vi "configuration UI.vi"() -> ()   [LabVIEW 2013, in "EIP Tags editor node.lvclass"]
uses:
  EIP Tags editor node.lvclass
  <vilib>/NI/Configuration Framework/Node/NodeRef.ctl
  <vilib>/NI/Configuration Framework/Node/NISE_CEF_Node.lvclass
  <vilib>/NI/AMC/Message Queue.ctl
  <vilib>/NI/AMC/Message.ctl
  <vilib>/NI/Tools/Keyed Array/KeyedArray.ctl
  <vilib>/NI/Configuration Framework/Node/UserEventRef.ctl
  <vilib>/NI/Configuration Framework/Controls/EventCluster.ctl
  <vilib>/NI/DCAF UI Toolkit/Controls/Configure.ctl
  <vilib>/NI/DCAF UI Toolkit/Controls/Add.ctl
  <vilib>/NI/DCAF UI Toolkit/Controls/Remove.ctl
  <vilib>/NI/DCAF UI Toolkit/Controls/Import.ctl
  <vilib>/Utility/miscctls.llb/LVPositionTypeDef.ctl
  <vilib>/NI/DCAF/Tag Editor Core/Configuration Editor/Classes/Engine Parent/Engine Parent Editor Node.lvclass
  <vilib>/NI/Tag Bus/tag/tag descriptor.lvclass
  <vilib>/NI/Tag Bus/tag/Data Type.ctl
  <vilib>/NI/Module Execution Interface/Engine Configuration/engine configuration.lvclass
  configuration/EIP Tags Configuration.lvclass
  <vilib>/NI/Tag Bus/tag/tag descriptor.lvclass/tag descriptor.ctl
  EIP Tags editor node.lvclass/EIP Tags editor node.ctl
  configuration/eip tag definition.ctl
  configuration/eip tag types.ctl
  <vilib>/NI/Configuration Framework/serializable configuration/NISE_CEF_serializable configuration.lvclass/NISE_CEF_serializable configuration.ctl
  <vilib>/NI/Tag Bus/tag/write tag name.vi
  <vilib>/NI/Tag Bus/tag/write data type.vi
  <vilib>/NI/DCAF/Tag Editor Core/Configuration Editor/Classes/Module editor node/Read Module Configuration.vi
  <vilib>/Utility/LVClass/Get LV Class Name.vi
  <vilib>/NI/Configuration Framework/error generator/NISE_error generator.vi
  <vilib>/NI/Tag Bus Module Framework/module configuration/TBM module configuration.lvclass
  <vilib>/NI/Configuration Framework/NISE_CEF_TreeControl.lvlib
  <vilib>/NI/DCAF/Tag Editor Core/Configuration Editor/Classes/Module editor node/module editor node.lvclass
  <vilib>/NI/Configuration Framework/serializable configuration/NISE_CEF_serializable configuration.lvclass
  <vilib>/NI/DCAF UI Toolkit/Controls/DCAF UI Elements.lvlib
  <vilib>/NI/Tools/Keyed Array/Tools_KeyedArray.lvlib
  <vilib>/NI/AMC/AMC.lvlib
panel:
  in  "Top Level Tab Control":enum32{"EIP Tags", "Channels"}(tab)
  in  "EIP tags":i32(listbox)
  in  "Add EIPT":T1
  in  "Remove EIPT":T2
  in  "configure EIPT":T3
  in  "generate from csv":T4
  in  "settings":T3
  in  "channel":i32(listbox)
  in  "Add Button":T1
  in  "Remove Button":T2
  in  "hidden_add":bool
  in  "user event":T5
  in  "main queue":T6
  in  "node ref":T7
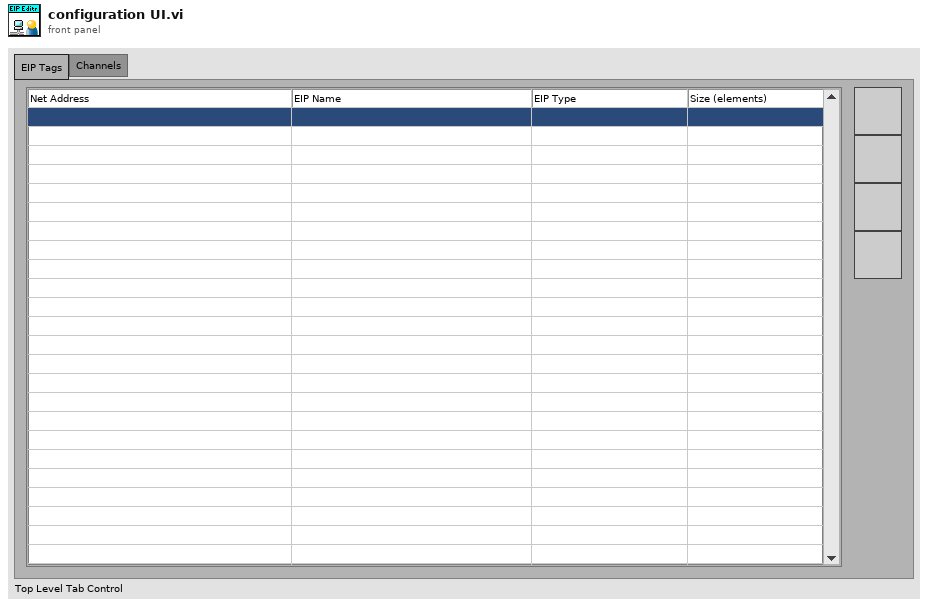
[diagram p1: front panel]
types:
  T1 = typedef "DCAF UI Elements.lvlib/Add.ctl" = bool
  T2 = typedef "DCAF UI Elements.lvlib/Remove.ctl" = bool
  T3 = typedef "DCAF UI Elements.lvlib/Configure.ctl" = bool
  T4 = typedef "DCAF UI Elements.lvlib/Import.ctl" = bool
  T5 = typedef "NISE_CEF_Node.lvclass/UserEventRef.ctl" = refnum<user-event>
  T6 = typedef "AMC.lvlib/Message Queue.ctl" = refnum<queue>
  T7 = typedef "NISE_CEF_Node.lvclass/NodeRef.ctl" = refnum<data-value>
  T8 = typedef "LVPositionTypeDef.ctl" = cluster{"Left":i32, "Top":i32}
  T9 = typedef "NISE_CEF_TreeControl.lvlib/EventCluster.ctl" = cluster{"command":string, "data":string}
  T10 = typedef "tag bus.lvlib/tag descriptor.lvclass/Data Type.ctl" = enum16{"Double", "Single", "I64", "I32", "I16", "I8", "U64", "U32", "U16", "U8", "Boolean", "String", "Array of Double", "Array of Single", "Array of I64", "Array of I32", "Array of I16", "Array of I8", "Array of U64", "Array of U32", "Array of U16", "Array of U8", "Array of Boolean", "Array of String"}
  T11 = typedef "EIP Tags Configuration.lvclass/eip tag definition.ctl" = cluster{"eip tag types":T12, "unique tag name":string, "Number of Elements":u32}
  T12 = typedef "EIP Tags Configuration.lvclass/eip tag types.ctl" = enum16{"SINT", "INT", "DINT", "REAL", "BOOL", "STRING"}
  T13 = typedef "EIP Tags editor node.lvclass/table line.ctl" = cluster{"eip channel":refnum<class "EIP Tags Channel.lvclass">, "tag name":string}
  T14 = typedef "LVPoint32TypeDef.ctl" = cluster{"Horizontal":i32, "Vertical":i32}
  T15 = typedef "LVRowAndColumnTypeDef.ctl" = cluster{"Row":i32, "Column":i32}
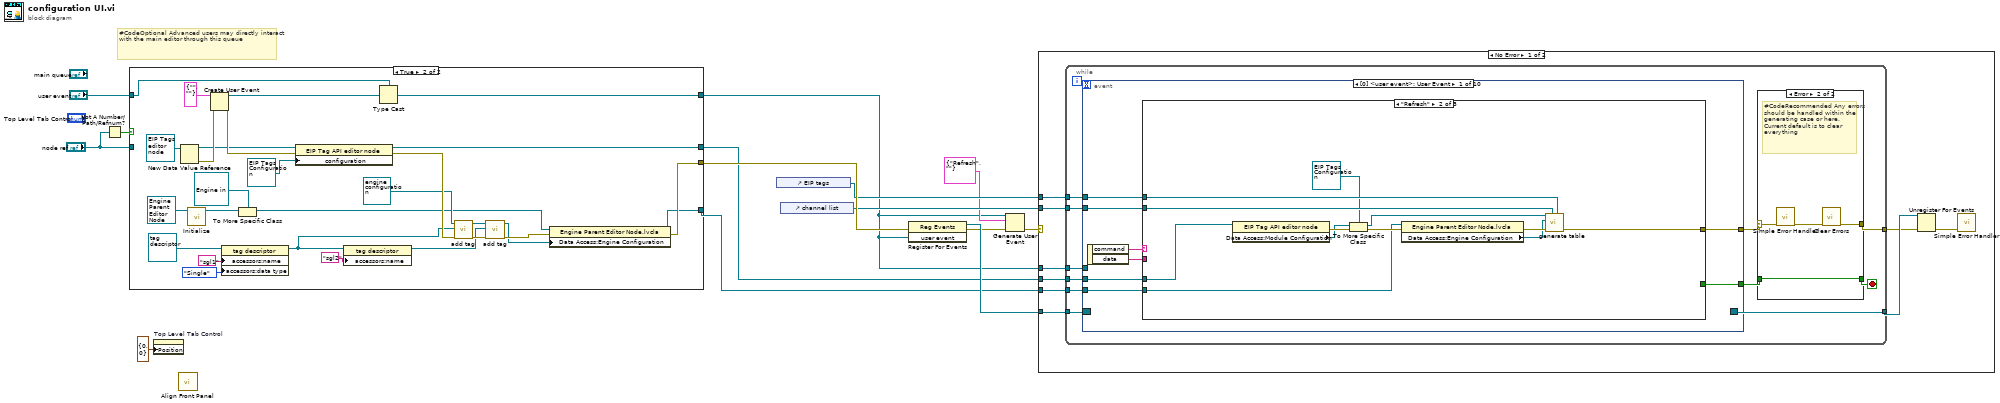
[diagram p0: block diagram]
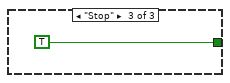
[diagram p4: hidden frame]
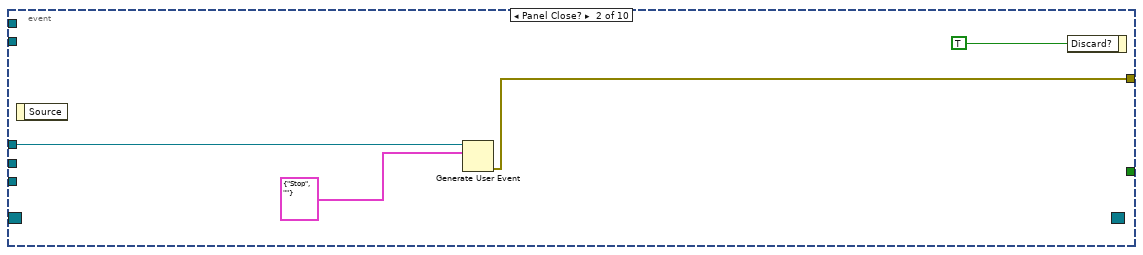
[diagram p5: hidden frame]
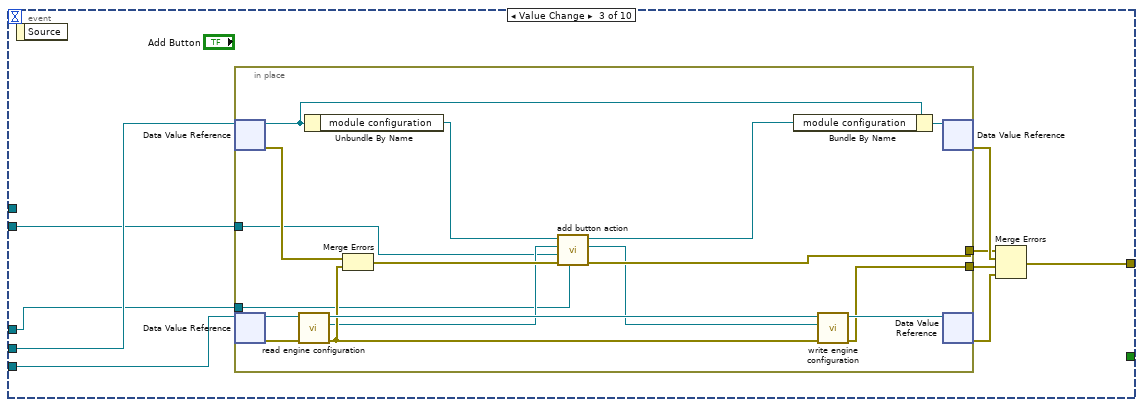
[diagram p6: hidden frame]
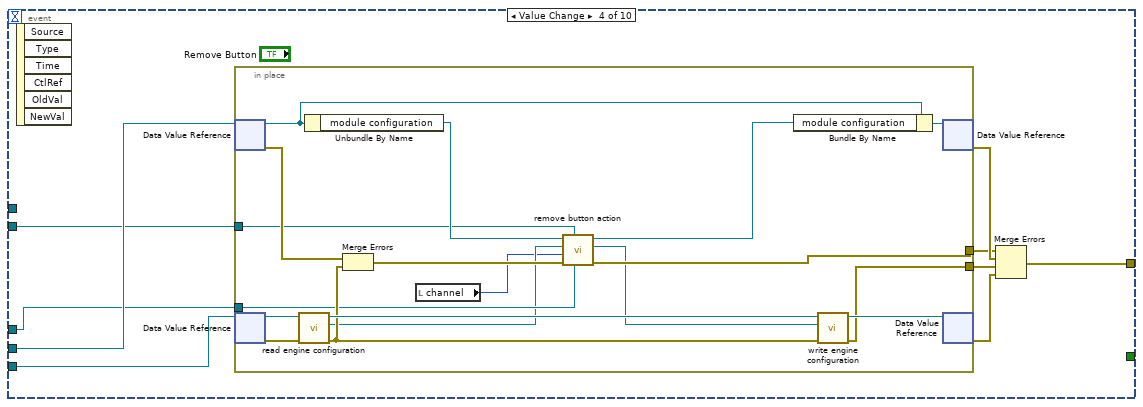
[diagram p7: hidden frame]
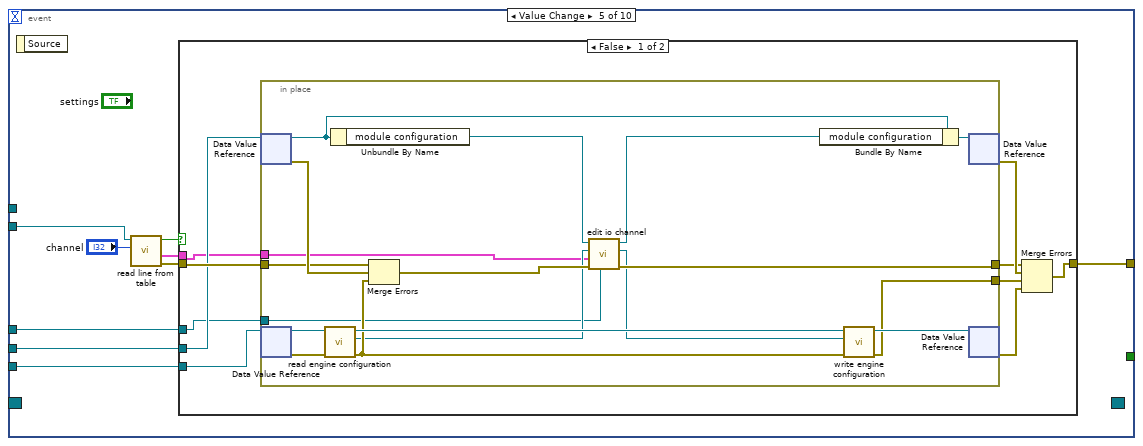
[diagram p8: hidden frame]
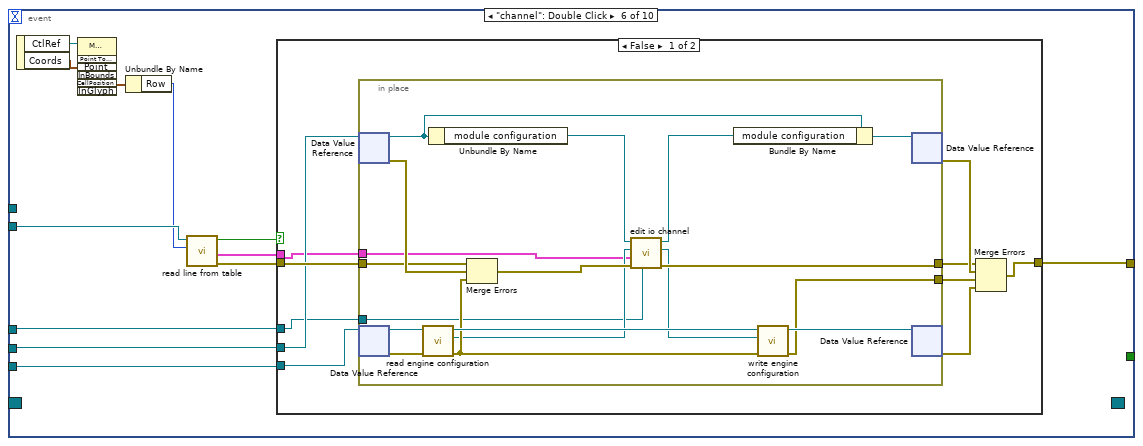
[diagram p10: hidden frame]
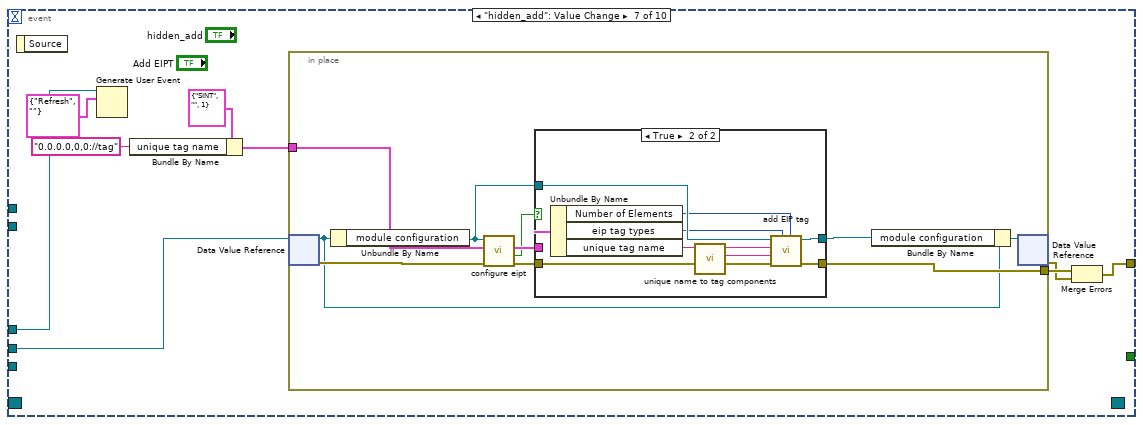
[diagram p12: hidden frame]
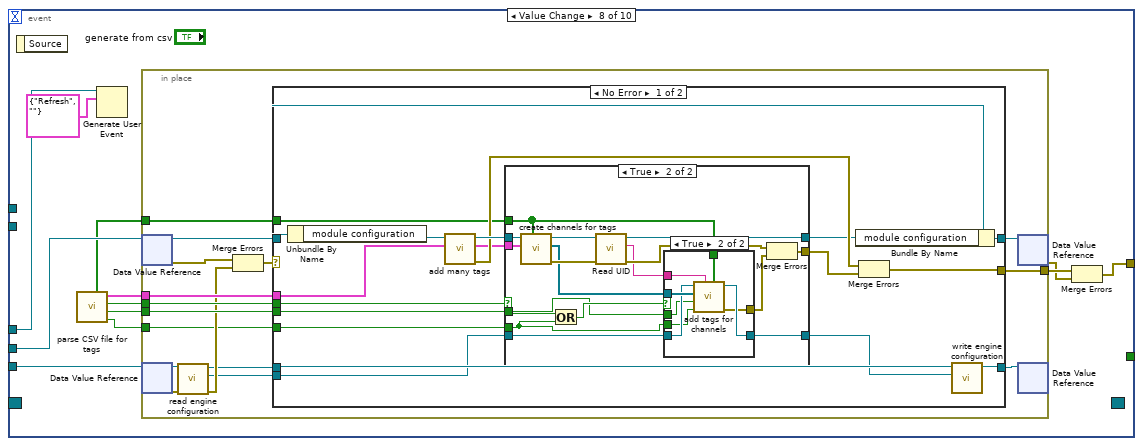
[diagram p14: hidden frame]
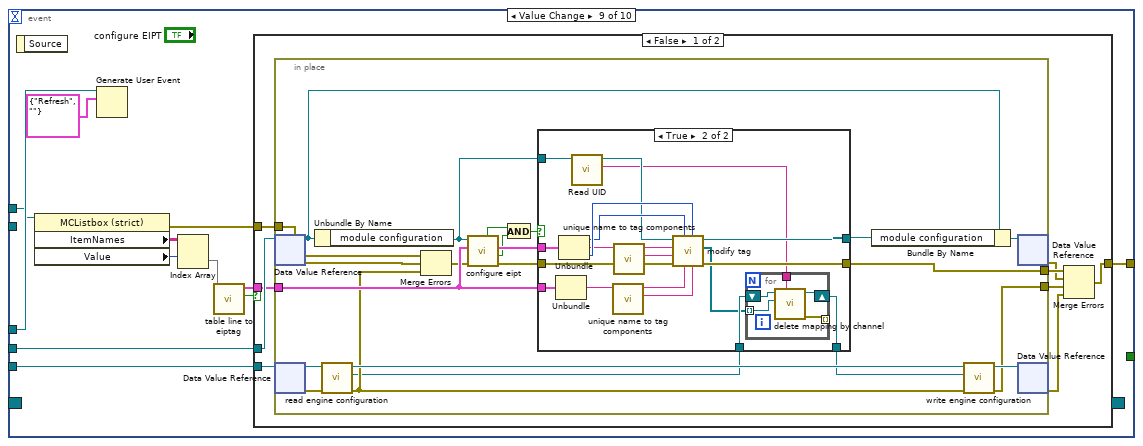
[diagram p18: hidden frame]
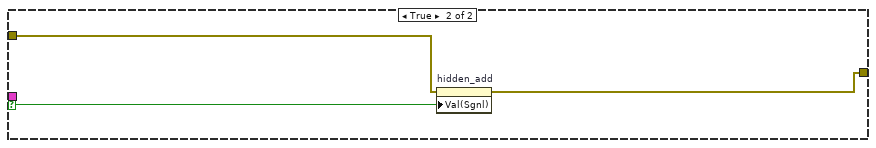
[diagram p20: hidden frame]
diagram:
  # "#CodeOptional Advanced users may directly interact with the main editor through this queue"
  n1 = Not A Number/Path/Refnum?(number/path/refnum="node ref") -> (NaN/Path/Refnum?=w13:bool)
  n2 = case shown="True" w13 {
    tunnel: "user event" -> [w21 w28]
    tunnel: [w21 w29] -> w4
    tunnel: "node ref" -> [w19 _]
    tunnel: [w18 w44] -> w9
    tunnel: [w17 w25] -> w11
    tunnel: [w16 w23] -> w8
    frame False {
      n3 = call <vilib>:"locate engine.vi"("component"=w19) -> ("error out"=w15:errorcluster, "engine"=w16:refnum<data-value>)  [unwired: 9 in]
      n4 = To More Specific Class(target class=refnum<data-value> refnum ("data value reference"), reference=w19, error in=w15) -> (specific class reference=w18:refnum<data-value>, error out=w17:errorcluster)
    }
    frame True {
      n5 = New Data Value Reference(data value=refnum<class "EIP Tags editor node.lvclass"> refnum ("tag bus configurable plugin editor node")) -> (data value reference=w43:refnum<data-value>, error out=w46:errorcluster)  [unwired: 1 in]
      n6 = call-dynamic "Initialize.vi"("Engine in"=refnum<class "Engine Parent Editor Node.lvclass"> refnum) -> ("data value reference"=w42:T7)  [unwired: 8 in, 2 out]
      n7 = Create User Event(user event datatype=T9 {"command"="", "data"=""} ("event data"), error in=w46) -> (user event=w48:refnum<user-event>, error out=w45:errorcluster)
      n8 = property class="tag descriptor"(reference=refnum<class "tag descriptor.lvclass"> refnum ("tag descriptor"), "accessors:name"="sgl1" ("name"), "accessors:data type"=Data_Type."Single" ("data type")) -> (reference out=w30:refnum<class "tag descriptor.lvclass">)  [unwired: 1 in, 1 out]
      n9 = To More Specific Class(target class=refnum<data-value> refnum ("data value reference"), reference=w42) -> (specific class reference=w24:refnum<data-value>)  [unwired: 1 in, 1 out]
      n10 = property class="EIP Tag API editor node"(reference=w43, error in=w45, "configuration"=refnum<class "EIP Tags Configuration.lvclass"> refnum ("tag bus configurable plugin module configuration")) -> (reference out=w44:refnum<data-value>, error out=w36:errorcluster)
      n11 = property class="tag descriptor"(reference=w30, "accessors:name"="sgl2" ("name")) -> (reference out=w31:refnum<class "tag descriptor.lvclass">)  [unwired: 1 in, 1 out]
      n12 = Type Cast(type=w28, x=w48) -> (*(type *) &x=w29:T5)
      n13 = call <vilib>:"add tag.vi"("error in"=w36, "tag descriptor"=w30, "engine configuration in"=refnum<class "engine configuration.lvclass"> refnum ("Engine Configuration")) -> ("error out"=w34:errorcluster, "engine configuration out"=w33:refnum<class "engine configuration.lvclass">)  [unwired: 7 in]
      n14 = call <vilib>:"add tag.vi"("error in"=w34, "tag descriptor"=w31, "engine configuration in"=w33) -> ("error out"=w32:errorcluster, "engine configuration out"=w22:refnum<class "engine configuration.lvclass">)  [unwired: 7 in]
      n15 = property class="Engine Parent Editor Node.lvcla"(reference=w24, error in=w32, "Data Access:Engine Configuration"=w22) -> (reference out=w23:refnum<data-value>, error out=w25:errorcluster)
    }
  }
  n16 = property on="Top Level Tab Control" class="TabCtl (strict)"("Position"=T8 {"Left"=0, "Top"=0}) -> ()  [unwired: 2 in, 2 out]
  n17 = call <vilib>:"Align Front Panel.vi"() -> ()  [unwired: 10 in, 2 out]
  n18 = control-ref of="EIP tags"() -> (w6:refnum<vi>)
  n19 = control-ref of="channel list"() -> (w7:refnum<vi>)
  n20 = register-events(error in=w11, w4) -> (reference out=w14:refnum<event-registration>, error out=w3:errorcluster)  [unwired: 1 in]
  n21 = Generate User Event(user event=w4, event data cluster=T9 {"command"="Refresh", "data"=""} ("event data"), error in=w3) -> (error out=w2:errorcluster)  [unwired: 1 in, 1 out]
  n22 = case shown="No Error" w2 {
    tunnel: w14 -> [w58 _]
    tunnel: w9 -> [w55 _]
    tunnel: w8 -> [w54 _]
    tunnel: w7 -> [w52 _]
    tunnel: w6 -> [w51 _]
    tunnel: w4 -> [w50 _]
    frame No Error {
      n23 = while {
        tunnel: w58 -> [w69]
        tunnel: [w68] -> w57
        tunnel: w55 -> [w64]
        tunnel: w54 -> [w63]
        tunnel: w50 -> [w62]
        tunnel: w52 -> [w60]
        tunnel: w51 -> [w59]
        tunnel: [w65] -> w56
        stop <- w67 stop-if-true
        n24 = event shown="[0] <user event>: User Event" {
          selector: w69 -> [_ _ _ _ _ _ _ _ _ _]
          dyn-events: [_ _ _ _ _ _ _ _ _ _] -> w68
          timeout: _ -> [_ _ _ _ _ _ _ _ _ _]
          tunnel: [w83 _ _ _ _ _ _ _ _ _] -> w66
          tunnel: [w78 w97 w105 w131 w162 w195 w234 w271 w348 w418] -> w61
          tunnel: w64 -> [w81 _ w103 w129 w154 w193 w235 w272 w349 w416]
          tunnel: w63 -> [w80 _ w104 w130 w155 w192 _ w266 w341 w417]
          tunnel: w62 -> [_ w99 w101 w127 w158 w194 w238 w273 w350 w425]
          tunnel: w60 -> [w77 _ w102 w128 w156 w203 _ _ _ _]
          tunnel: w59 -> [w76 _ _ _ _ _ _ _ w347 w428]
          event User Event {
            n25 = event-data() -> ("command"=w82:string, "data"=w79:string)  [unwired: 1 in]
            n26 = case shown="\"Refresh\"" w82 {
              tunnel: [_ _ TRUE] -> w83
              tunnel: w81 -> [_ w90 _]
              tunnel: w80 -> [_ w85 _]
              tunnel: w79 -> [_ _ _]
              tunnel: [_ w95 _] -> w78
              tunnel: w77 -> [_ w94 _]
              tunnel: w76 -> [_ w93 _]
              frame Default {
              }
              frame "Refresh" {
                n27 = property class="EIP Tag API editor node"(reference=w90) -> (error out=w91:errorcluster, "Data Access:Module Configuration"=w88:refnum<class "TBM module configuration.lvclass">)  [unwired: 1 in, 1 out]
                n28 = To More Specific Class(target class=refnum<class "EIP Tags Configuration.lvclass"> refnum ("tag bus configurable plugin module configuration"), reference=w88, error in=w91) -> (specific class reference=w86:refnum<class "EIP Tags Configuration.lvclass">, error out=w89:errorcluster)
                n29 = property class="Engine Parent Editor Node.lvcla"(reference=w85, error in=w89) -> (error out=w92:errorcluster, "Data Access:Engine Configuration"=w84:refnum<class "engine configuration.lvclass">)  [unwired: 1 out]
                n30 = call "generate table.vi"("assemblies"=w93, "table"=w94, "error in"=w92, "engine configuration in"=w84, "EthernetIP configuration in"=w86) -> ("error out"=w95:errorcluster)  [unwired: 6 in]
              }
              frame "Stop" {
              }
            }
          }
          event Panel Close? {
            n31 = event-data() -> ()  [unwired: 1 in, 1 out]
            n32 = Generate User Event(user event=w99, event data cluster=T9 {"command"="Stop", "data"=""} ("event data")) -> (error out=w97:errorcluster)  [unwired: 2 in, 1 out]
            n33 = event-data("Discard?"=TRUE) -> ()  [unwired: 1 in, 1 out]
          }
          event Value Change {
            n34 = event-data() -> ()  [unwired: 1 in, 1 out]
            n35 = in-place {
              in-place-border: [w116] -> w106
              in-place-border: [w122] -> w109
              in-place-border: w102 -> [w111]
              in-place-border: w101 -> [w110]
              n36 = in-place-dvr #1(w103) -> (w126:refnum<class "EIP Tags editor node.lvclass">, w124:errorcluster)
              n37 = in-place-dvr #2(w104) -> (w121:refnum<class "Engine Parent Editor Node.lvclass">, w120:errorcluster)
              n38 = call <vilib>:"read engine configuration.vi"("error in"=w120, "Engine Parent Editor Node in"=w121) -> ("error out"=w118:errorcluster, "engine configuration"=w113:refnum<class "engine configuration.lvclass">, "Engine Parent Editor Node out"=w119:refnum<class "Engine Parent Editor Node.lvclass">)  [unwired: 7 in]
              n39 = Unbundle By Name(w126) -> ("module configuration"=w114:refnum<class "EIP Tags Configuration.lvclass">)
              n40 = Merge Errors(w124, w118) -> (w117:errorcluster)
              n41 = call "add button action.vi"("user event"=w110, "error in"=w117, "channel list"=w111, "Engine Configuration"=w113, "EIP Tags Configuration in"=w114) -> ("error out"=w116:errorcluster, "Engine Configuration out"=w112:refnum<class "engine configuration.lvclass">, "module configuration out"=w115:refnum<class "EIP Tags Configuration.lvclass">)  [unwired: 4 in]
              n42 = Bundle By Name(cluster=w126, "module configuration"=w115) -> (w125:refnum<class "EIP Tags editor node.lvclass">)
              n43 = call <vilib>:"write engine configuration.vi"("error in"=w118, "engine configuration"=w112, "Engine Parent Editor Node in"=w119) -> ("error out"=w122:errorcluster, "Engine Parent Editor Node out"=w123:refnum<class "Engine Parent Editor Node.lvclass">)  [unwired: 7 in]
              n44 = in-place-dvr #1(w125) -> (w108:errorcluster)  [unwired: 1 out]
              n45 = in-place-dvr #2(w123) -> (w107:errorcluster)  [unwired: 1 out]
            }
            n46 = Merge Errors(w106, w108, w109, w107) -> (w105:errorcluster)
          }
          event Value Change {
            n47 = event-data() -> ()  [unwired: 1 in, 6 out]
            n48 = in-place {
              in-place-border: [w143] -> w132
              in-place-border: [w149] -> w135
              in-place-border: w128 -> [w139]
              in-place-border: w127 -> [w142]
              n49 = in-place-dvr #3(w129) -> (w153:refnum<class "EIP Tags editor node.lvclass">, w151:errorcluster)
              n50 = in-place-dvr #4(w130) -> (w148:refnum<class "Engine Parent Editor Node.lvclass">, w147:errorcluster)
              n51 = call <vilib>:"read engine configuration.vi"("error in"=w147, "Engine Parent Editor Node in"=w148) -> ("error out"=w145:errorcluster, "engine configuration"=w138:refnum<class "engine configuration.lvclass">, "Engine Parent Editor Node out"=w146:refnum<class "Engine Parent Editor Node.lvclass">)  [unwired: 7 in]
              n52 = Unbundle By Name(w153) -> ("module configuration"=w140:refnum<class "EIP Tags Configuration.lvclass">)
              n53 = Merge Errors(w151, w145) -> (w144:errorcluster)
              n54 = local read "channel"() -> (w136:i32)
              n55 = call "remove button action.vi"("user event"=w142, "channel list"=w139, "error in"=w144, "channel"=w136, "Engine Configuration in"=w138, "EIP Tags Configuration in"=w140) -> ("error out"=w143:errorcluster, "Engine Configuration out"=w137:refnum<class "engine configuration.lvclass">, "EIP Tags Configuration out"=w141:refnum<class "EIP Tags Configuration.lvclass">)  [unwired: 3 in]
              n56 = Bundle By Name(cluster=w153, "module configuration"=w141) -> (w152:refnum<class "EIP Tags editor node.lvclass">)
              n57 = call <vilib>:"write engine configuration.vi"("error in"=w145, "engine configuration"=w137, "Engine Parent Editor Node in"=w146) -> ("error out"=w149:errorcluster, "Engine Parent Editor Node out"=w150:refnum<class "Engine Parent Editor Node.lvclass">)  [unwired: 7 in]
              n58 = in-place-dvr #3(w152) -> (w134:errorcluster)  [unwired: 1 out]
              n59 = in-place-dvr #4(w150) -> (w133:errorcluster)  [unwired: 1 out]
            }
            n60 = Merge Errors(w132, w134, w135, w133) -> (w131:errorcluster)
          }
          event Value Change {
            n61 = event-data() -> ()  [unwired: 1 in, 1 out]
            n62 = call "read line from table.vi"("line number"="channel", "channels table"=w156) -> ("error out"=w161:errorcluster, "line"=w160:T13, "empty channel?"=w157:bool)  [unwired: 6 in, 1 out]
            n63 = case shown="False" w157 {
              tunnel: [w168 w191] -> w162
              tunnel: w161 -> [w167 w191]
              tunnel: w160 -> [w164 _]
              tunnel: w158 -> [w163 _]
              tunnel: w155 -> [w166 _]
              tunnel: w154 -> [w165 _]
              frame False {
                n64 = in-place {
                  in-place-border: [w179] -> w169
                  in-place-border: [w186] -> w172
                  in-place-border: w167 -> [w181]
                  in-place-border: w164 -> [w174]
                  in-place-border: w163 -> [w173]
                  n65 = in-place-dvr #5(w165) -> (w190:refnum<class "EIP Tags editor node.lvclass">, w188:errorcluster)
                  n66 = in-place-dvr #6(w166) -> (w185:refnum<class "Engine Parent Editor Node.lvclass">, w184:errorcluster)
                  n67 = call <vilib>:"read engine configuration.vi"("error in"=w184, "Engine Parent Editor Node in"=w185) -> ("error out"=w182:errorcluster, "engine configuration"=w175:refnum<class "engine configuration.lvclass">, "Engine Parent Editor Node out"=w183:refnum<class "Engine Parent Editor Node.lvclass">)  [unwired: 7 in]
                  n68 = Unbundle By Name(w190) -> ("module configuration"=w178:refnum<class "EIP Tags Configuration.lvclass">)
                  n69 = Merge Errors(w181, w188, w182) -> (w180:errorcluster)
                  n70 = call "edit io channel.vi"("user event"=w173, "error in"=w180, "line"=w174, "engine configuration in"=w175, "EthernetIP configuration in"=w178) -> ("error out"=w179:errorcluster, "engine configuration out"=w176:refnum<class "engine configuration.lvclass">, "EthernetIP configuration out"=w177:refnum<class "EIP Tags Configuration.lvclass">)  [unwired: 4 in]
                  n71 = Bundle By Name(cluster=w190, "module configuration"=w177) -> (w189:refnum<class "EIP Tags editor node.lvclass">)
                  n72 = call <vilib>:"write engine configuration.vi"("error in"=w182, "engine configuration"=w176, "Engine Parent Editor Node in"=w183) -> ("error out"=w186:errorcluster, "Engine Parent Editor Node out"=w187:refnum<class "Engine Parent Editor Node.lvclass">)  [unwired: 7 in]
                  n73 = in-place-dvr #5(w189) -> (w171:errorcluster)  [unwired: 1 out]
                  n74 = in-place-dvr #6(w187) -> (w170:errorcluster)  [unwired: 1 out]
                }
                n75 = Merge Errors(w169, w171, w172, w170) -> (w168:errorcluster)
              }
              frame True {
              }
            }
          }
          event "channel": Double Click {
            n76 = event-data() -> ("CtlRef"=w202:refnum<vi>, "Coords"=w201:T14)  [unwired: 1 in]
            n77 = invoke class="MCListbox (strict)" method="Point To Row Column"(reference=w202, "Point"=w201) -> ("CellPosition"=w200:T15)  [unwired: 5 in, 6 out]
            n78 = Unbundle By Name(w200) -> ("Row"=w199:i32)
            n79 = call "read line from table.vi"("line number"=w199, "channels table"=w203) -> ("error out"=w198:errorcluster, "line"=w197:T13, "empty channel?"=w196:bool)  [unwired: 6 in, 1 out]
            n80 = case shown="False" w196 {
              tunnel: [w209 w232] -> w195
              tunnel: w198 -> [w208 w232]
              tunnel: w197 -> [w205 _]
              tunnel: w194 -> [w204 _]
              tunnel: w192 -> [w207 _]
              tunnel: w193 -> [w206 _]
              frame False {
                n81 = in-place {
                  in-place-border: [w220] -> w210
                  in-place-border: [w227] -> w213
                  in-place-border: w208 -> [w222]
                  in-place-border: w205 -> [w215]
                  in-place-border: w204 -> [w214]
                  n82 = in-place-dvr #7(w206) -> (w231:refnum<class "EIP Tags editor node.lvclass">, w229:errorcluster)
                  n83 = in-place-dvr #8(w207) -> (w226:refnum<class "Engine Parent Editor Node.lvclass">, w225:errorcluster)
                  n84 = call <vilib>:"read engine configuration.vi"("error in"=w225, "Engine Parent Editor Node in"=w226) -> ("error out"=w223:errorcluster, "engine configuration"=w216:refnum<class "engine configuration.lvclass">, "Engine Parent Editor Node out"=w224:refnum<class "Engine Parent Editor Node.lvclass">)  [unwired: 7 in]
                  n85 = Unbundle By Name(w231) -> ("module configuration"=w219:refnum<class "EIP Tags Configuration.lvclass">)
                  n86 = Merge Errors(w222, w229, w223) -> (w221:errorcluster)
                  n87 = call "edit io channel.vi"("user event"=w214, "error in"=w221, "line"=w215, "engine configuration in"=w216, "EthernetIP configuration in"=w219) -> ("error out"=w220:errorcluster, "engine configuration out"=w217:refnum<class "engine configuration.lvclass">, "EthernetIP configuration out"=w218:refnum<class "EIP Tags Configuration.lvclass">)  [unwired: 4 in]
                  n88 = Bundle By Name(cluster=w231, "module configuration"=w218) -> (w230:refnum<class "EIP Tags editor node.lvclass">)
                  n89 = call <vilib>:"write engine configuration.vi"("error in"=w223, "engine configuration"=w217, "Engine Parent Editor Node in"=w224) -> ("error out"=w227:errorcluster, "Engine Parent Editor Node out"=w228:refnum<class "Engine Parent Editor Node.lvclass">)  [unwired: 7 in]
                  n90 = in-place-dvr #7(w230) -> (w212:errorcluster)  [unwired: 1 out]
                  n91 = in-place-dvr #8(w228) -> (w211:errorcluster)  [unwired: 1 out]
                }
                n92 = Merge Errors(w210, w212, w213, w211) -> (w209:errorcluster)
              }
              frame True {
              }
            }
          }
          event "hidden_add": Value Change {
            n93 = event-data() -> ()  [unwired: 1 in, 1 out]
            n94 = Generate User Event(user event=w238, event data cluster=T9 {"command"="Refresh", "data"=""} ("event data")) -> ()  [unwired: 2 in, 2 out]
            n95 = Bundle By Name(cluster=T11 {"eip tag types"=enum."SINT", "unique tag name"="", "Number of Elements"=1} ("tag spec"), "unique tag name"="0.0.0.0,0,0://tag") -> (w240:T11)
            n96 = in-place {
              in-place-border: [w250] -> w241
              in-place-border: w240 -> [w247]
              n97 = in-place-dvr #9(w235) -> (w244:refnum<class "EIP Tags editor node.lvclass">, w246:errorcluster)
              n98 = Unbundle By Name(w244) -> ("module configuration"=w242:refnum<class "EIP Tags Configuration.lvclass">)
              n99 = call "configure eipt.vi"("error in"=w246, "tag definition in"=w247, "EthernetIP configuration"=w242) -> ("error out"=w251:errorcluster, "success"=w248:bool, "tag definition out"=w249:T11)  [unwired: 5 in, 1 out]
              n100 = case shown="True" w248 {
                tunnel: w251 -> [w252 w263]
                tunnel: [w252 w262] -> w250
                tunnel: [w253 w261] -> w243
                tunnel: w242 -> [w253 w260]
                tunnel: w249 -> [_ w259]
                frame False {
                }
                frame True {
                  n101 = Unbundle By Name(w259) -> ("Number of Elements"=w257:u32, "eip tag types"=w258:T12, "unique tag name"=w256:string)
                  n102 = call "unique name to tag components.vi"("unique name"=w256) -> ("Tag Name"=w254:string, "Network Path"=w255:string)  [unwired: 9 in]
                  n103 = call "add EIP tag.vi"("Number of Elements"=w257, "eip tag types"=w258, "error in"=w263, "Tag Name"=w254, "Network Path"=w255, "EIP Tags configuration in"=w260) -> ("error out"=w262:errorcluster, "EIP Tags configuration out"=w261:refnum<class "EIP Tags Configuration.lvclass">)  [unwired: 4 in]
                }
              }
              n104 = Bundle By Name(cluster=w244, "module configuration"=w243) -> (w245:refnum<class "EIP Tags editor node.lvclass">)
              n105 = in-place-dvr #9(w245) -> (w233:errorcluster)  [unwired: 1 out]
            }
            n106 = Merge Errors(w241, w233) -> (w234:errorcluster)
          }
          event Value Change {
            n107 = event-data() -> ()  [unwired: 1 in, 1 out]
            n108 = call "parse CSV file for tags.vi"() -> ("create input tags?"=w264:bool, "create output tags?"=w267:bool, "create channels?"=w268:bool, "tags"=w269:T11[], "outputs?"=w265:bool[])  [unwired: 7 in]
            n109 = Generate User Event(user event=w273, event data cluster=T9 {"command"="Refresh", "data"=""} ("event data")) -> ()  [unwired: 2 in, 2 out]
            n110 = in-place {
              in-place-border: [w291] -> w275
              in-place-border: w269 -> [w287]
              in-place-border: w268 -> [w286]
              in-place-border: w267 -> [w285]
              in-place-border: w265 -> [w277]
              in-place-border: w264 -> [w276]
              n111 = in-place-dvr #10(w272) -> (w289:refnum<class "EIP Tags editor node.lvclass">, w288:errorcluster)
              n112 = in-place-dvr #11(w266) -> (w283:refnum<class "Engine Parent Editor Node.lvclass">, w282:errorcluster)
              n113 = call <vilib>:"read engine configuration.vi"("error in"=w282, "Engine Parent Editor Node in"=w283) -> ("error out"=w281:errorcluster, "engine configuration"=w278:refnum<class "engine configuration.lvclass">, "Engine Parent Editor Node out"=w279:refnum<class "Engine Parent Editor Node.lvclass">)  [unwired: 7 in]
              n114 = Merge Errors(w288, w281) -> (w284:errorcluster)
              n115 = case shown="No Error" w284 {
                selector: w284 -> [_ w338]
                tunnel: [w302 w338] -> w291
                tunnel: [w309 w339] -> w290
                tunnel: w289 -> [w308 w339]
                tunnel: w287 -> [w306 _]
                tunnel: w286 -> [w300 _]
                tunnel: w285 -> [w298 _]
                tunnel: [w305 w337] -> w280
                tunnel: w279 -> [w304 w337]
                tunnel: w278 -> [w296 _]
                tunnel: w277 -> [w293 _]
                tunnel: w276 -> [w292 _]
                frame No Error {
                  n116 = Unbundle By Name(w308) -> ("module configuration"=w307:refnum<class "EIP Tags Configuration.lvclass">)
                  n117 = call "add many tags.vi"("tags"=w306, "EIP Tags Configuration in"=w307) -> ("error out"=w301:errorcluster, "Array"=w295:T11[], "EIP Tags Configuration out"=w303:refnum<class "EIP Tags Configuration.lvclass">)  [unwired: 7 in]
                  n118 = case shown="True" w300 {
                    tunnel: w303 -> [w311 w327]
                    tunnel: [w311 w317] -> w299
                    tunnel: w298 -> [_ w313]
                    tunnel: [w310 w324] -> w297
                    tunnel: w296 -> [w310 w323]
                    tunnel: w295 -> [_ w326]
                    tunnel: [_ w321] -> w294
                    tunnel: w293 -> [_ w314]
                    tunnel: w292 -> [_ w312]
                    frame False {
                    }
                    frame True {
                      n119 = call "create channels for tags.vi"("outputs?"=w314, "tags in"=w326, "EIP Tags Configuration in"=w327) -> ("error out"=w325:errorcluster, "channels"=w320:refnum<class "EIP Tags Channel.lvclass">[], "EIP Tags Configuration out"=w318:refnum<class "EIP Tags Configuration.lvclass">)  [unwired: 6 in]
                      n120 = Or(x=w313, y=w312) -> (x .or. y?=w315:bool)
                      n121 = call <vilib>:"Read UID.vi"("error in"=w325, "configuration in"=w318) -> ("error out"=w319:errorcluster, "instance id"=w316:string, "configuration out"=w317:refnum<class "EIP Tags Configuration.lvclass">)  [unwired: 7 in]
                      n122 = case shown="True" w315 {
                        tunnel: [w328 w335] -> w324
                        tunnel: w323 -> [w328 w334]
                        tunnel: [_ w333] -> w322
                        tunnel: w320 -> [_ w336]
                        tunnel: w316 -> [_ w332]
                        tunnel: w314 -> [_ w331]
                        tunnel: w313 -> [_ w330]
                        tunnel: w312 -> [_ w329]
                        frame False {
                        }
                        frame True {
                          n123 = call "add tags for channels.vi"("outputs?"=w331, "module instance"=w332, "create input tags?"=w329, "create output tags?"=w330, "channels"=w336, "engine configuration in"=w334) -> ("error IO"=w333:errorcluster, "engine configuration out"=w335:refnum<class "engine configuration.lvclass">)  [unwired: 4 in]
                        }
                      }
                      n124 = Merge Errors(w319, w322) -> (w321:errorcluster)
                    }
                  }
                  n125 = Bundle By Name(cluster=w308, "module configuration"=w299) -> (w309:refnum<class "EIP Tags editor node.lvclass">)
                  n126 = Merge Errors(w301, w294) -> (w302:errorcluster)
                  n127 = call <vilib>:"write engine configuration.vi"("engine configuration"=w297, "Engine Parent Editor Node in"=w304) -> ("Engine Parent Editor Node out"=w305:refnum<class "Engine Parent Editor Node.lvclass">)  [unwired: 8 in, 1 out]
                }
                frame Error {
                }
              }
              n128 = in-place-dvr #10(w290) -> (w270:errorcluster)  [unwired: 1 out]
              n129 = in-place-dvr #11(w280) -> ()  [unwired: 2 out]
            }
            n130 = Merge Errors(w275, w270) -> (w271:errorcluster)
          }
          event Value Change {
            n131 = event-data() -> ()  [unwired: 1 in, 1 out]
            n132 = property class="MCListbox (strict)"(reference=w347) -> (error out=w340:errorcluster, "ItemNames"=w346:string[][], "Value"=w345:i32)  [unwired: 1 in, 1 out]
            n133 = Generate User Event(user event=w350, event data cluster=T9 {"command"="Refresh", "data"=""} ("event data")) -> ()  [unwired: 2 in, 2 out]
            n134 = Index Array(array=w346, index (row)=w345) -> (element=w344:string[])  [unwired: 1 in]
            n135 = call "table line to eiptag.vi"("line strings"=w344) -> ("invalid?"=w343:bool, "tag"=w342:T11)  [unwired: 9 in]
            n136 = case shown="False" w343 {
              selector: w343 -> [_ w412]
              tunnel: w349 -> [w359 _]
              tunnel: [w358 w411] -> w348
              tunnel: w342 -> [w356 _]
              tunnel: w341 -> [w355 _]
              tunnel: w340 -> [w352 w410]
              frame False {
                n137 = in-place {
                  in-place-border: [w381] -> w360
                  in-place-border: w356 -> [w371]
                  in-place-border: [w364] -> w353
                  in-place-border: w352 -> [w361]
                  n138 = in-place-dvr #12(w359) -> (w377:refnum<class "EIP Tags editor node.lvclass">, w379:errorcluster)
                  n139 = in-place-dvr #13(w355) -> (w370:refnum<class "Engine Parent Editor Node.lvclass">, w369:errorcluster)
                  n140 = Unbundle By Name(w377) -> ("module configuration"=w375:refnum<class "EIP Tags Configuration.lvclass">)
                  n141 = call <vilib>:"read engine configuration.vi"("error in"=w369, "Engine Parent Editor Node in"=w370) -> ("error out"=w365:errorcluster, "engine configuration"=w363:refnum<class "engine configuration.lvclass">, "Engine Parent Editor Node out"=w366:refnum<class "Engine Parent Editor Node.lvclass">)  [unwired: 7 in]
                  n142 = Merge Errors(w361, w379, w365) -> (w368:errorcluster)
                  n143 = call "configure eipt.vi"("error in"=w368, "tag definition in"=w371, "EthernetIP configuration"=w375) -> ("error out"=w382:errorcluster, "success"=w372:bool, "tag definition out"=w380:T11, "changed"=w373:bool)  [unwired: 5 in]
                  n144 = And(x=w373, y=w372) -> (x .and. y?=w374:bool)
                  n145 = case shown="True" w374 {
                    tunnel: w382 -> [w384 w404]
                    tunnel: [w384 w403] -> w381
                    tunnel: [w385 w402] -> w376
                    tunnel: w375 -> [w385 w389]
                    tunnel: w380 -> [_ w400]
                    tunnel: w371 -> [_ w401]
                    tunnel: w363 -> [w383 w391]
                    tunnel: [w383 w390] -> w362
                    frame False {
                    }
                    frame True {
                      n146 = Unbundle(w401) -> ("unique tag name"=w394:string)  [unwired: 2 out]
                      n147 = Unbundle(w400) -> ("eip tag types"=w398:T12, "unique tag name"=w397:string, "Number of Elements"=w399:u32)
                      n148 = call <vilib>:"Read UID.vi"("configuration in"=w389) -> ("instance id"=w387:string, "configuration out"=w388:refnum<class "EIP Tags Configuration.lvclass">)  [unwired: 8 in, 1 out]
                      n149 = call "unique name to tag components.vi"("unique name"=w394) -> ("Tag Name"=w392:string, "Network Path"=w393:string)  [unwired: 9 in]
                      n150 = call "unique name to tag components.vi"("unique name"=w397) -> ("Tag Name"=w395:string, "Network Path"=w396:string)  [unwired: 9 in]
                      n151 = call "modify tag.vi"("original tag name"=w392, "Number of Elements"=w399, "original network path"=w393, "eip tag types"=w398, "error in"=w404, "Tag Name"=w395, "Network Path"=w396, "EIP Tags configuration in"=w388) -> ("error out"=w403:errorcluster, "removed channels"=w386:refnum<class "EIP Tags Channel.lvclass">[], "EIP Tags configuration out"=w402:refnum<class "EIP Tags Configuration.lvclass">)  [unwired: 1 in]
                      n152 = for {
                        shift-right: [w409] -> w390
                        shift-left: w391 -> [w408]
                        tunnel: [w407] -> _ mode=indexing
                        tunnel: w387 -> [w406]
                        tunnel: w386 -> [w405] mode=indexing
                        n153 = call <vilib>:"delete mapping by channel.vi"("owner ID"=w406, "channel"=w405, "engine configuration in"=w408) -> ("error out"=w407:errorcluster, "engine configuration out"=w409:refnum<class "engine configuration.lvclass">)  [unwired: 7 in]
                      }
                    }
                  }
                  n154 = Bundle By Name(cluster=w377, "module configuration"=w376) -> (w378:refnum<class "EIP Tags editor node.lvclass">)
                  n155 = call <vilib>:"write engine configuration.vi"("error in"=w365, "engine configuration"=w362, "Engine Parent Editor Node in"=w366) -> ("error out"=w364:errorcluster, "Engine Parent Editor Node out"=w367:refnum<class "Engine Parent Editor Node.lvclass">)  [unwired: 7 in]
                  n156 = in-place-dvr #12(w378) -> (w357:errorcluster)  [unwired: 1 out]
                  n157 = in-place-dvr #13(w367) -> (w354:errorcluster)  [unwired: 1 out]
                }
                n158 = Merge Errors(w360, w357, w353, w354) -> (w358:errorcluster)
              }
              frame True {
                n159 = property on="hidden_add" class="Bool (strict)"(error in=w410, "Val(Sgnl)"=w412) -> (error out=w411:errorcluster)  [unwired: 1 in, 1 out]
              }
            }
          }
          event Value Change {
            n160 = event-data() -> ()  [unwired: 1 in, 1 out]
            n161 = property class="MCListbox (strict)"(reference=w428) -> (error out=w415:errorcluster, "ItemNames"=w427:string[][])  [unwired: 1 in, 1 out]
            n162 = Generate User Event(user event=w425, event data cluster=T9 {"command"="Refresh", "data"=""} ("event data")) -> ()  [unwired: 2 in, 2 out]
            n163 = Index Array(array=w427, index (row)="EIP tags") -> (element=w423:string[])  [unwired: 1 in]
            n164 = Index Array(array=w423) -> (element #1=w414:string, element #2=w413:string)  [unwired: 2 in]
            n165 = in-place {
              in-place-border: [w429] -> w419
              in-place-border: [w446] -> w422
              in-place-border: w415 -> [w441]
              in-place-border: w414 -> [w439]
              in-place-border: w413 -> [w438]
              n166 = in-place-dvr #14(w416) -> (w450:refnum<class "EIP Tags editor node.lvclass">, w448:errorcluster)
              n167 = in-place-dvr #15(w417) -> (w445:refnum<class "Engine Parent Editor Node.lvclass">, w444:errorcluster)
              n168 = call <vilib>:"read engine configuration.vi"("error in"=w444, "Engine Parent Editor Node in"=w445) -> ("error out"=w442:errorcluster, "engine configuration"=w437:refnum<class "engine configuration.lvclass">, "Engine Parent Editor Node out"=w443:refnum<class "Engine Parent Editor Node.lvclass">)  [unwired: 7 in]
              n169 = Unbundle By Name(w450) -> ("module configuration"=w434:refnum<class "EIP Tags Configuration.lvclass">)
              n170 = Merge Errors(w441, w448, w442) -> (w440:errorcluster)
              n171 = call <vilib>:"Read UID.vi"("error in"=w440, "configuration in"=w434) -> ("error out"=w432:errorcluster, "instance id"=w430:string, "configuration out"=w431:refnum<class "EIP Tags Configuration.lvclass">)  [unwired: 7 in]
              n172 = call "delete EIP tag.vi"("error in"=w432, "Tag Name"=w438, "Network Path"=w439, "EIP Tags configuration in"=w431) -> ("error out"=w429:errorcluster, "removed channels"=w433:refnum<class "EIP Tags Channel.lvclass">[], "EIP Tags configuration out"=w435:refnum<class "EIP Tags Configuration.lvclass">)  [unwired: 5 in]
              n173 = for {
                shift-right: [w455] -> w436
                shift-left: w437 -> [w454]
                tunnel: w433 -> [w453] mode=indexing
                tunnel: [w452] -> _ mode=indexing
                tunnel: w430 -> [w451]
                n174 = call <vilib>:"delete mapping by channel.vi"("owner ID"=w451, "channel"=w453, "engine configuration in"=w454) -> ("error out"=w452:errorcluster, "engine configuration out"=w455:refnum<class "engine configuration.lvclass">)  [unwired: 7 in]
              }
              n175 = Bundle By Name(cluster=w450, "module configuration"=w435) -> (w449:refnum<class "EIP Tags editor node.lvclass">)
              n176 = call <vilib>:"write engine configuration.vi"("error in"=w442, "engine configuration"=w436, "Engine Parent Editor Node in"=w443) -> ("error out"=w446:errorcluster, "Engine Parent Editor Node out"=w447:refnum<class "Engine Parent Editor Node.lvclass">)  [unwired: 7 in]
              n177 = in-place-dvr #14(w449) -> (w421:errorcluster)  [unwired: 1 out]
              n178 = in-place-dvr #15(w447) -> (w420:errorcluster)  [unwired: 1 out]
            }
            n179 = Merge Errors(w419, w421, w422, w420) -> (w418:errorcluster)
          }
        }
        n180 = case shown="Error" w61 {
          selector: w61 -> [w70 w74]
          tunnel: [w71 w75] -> w67
          tunnel: w66 -> [w71 w75]
          tunnel: [w70 w72] -> w65
          frame No Error {
          }
          frame Error {
            # "#CodeRecommended Any errors should be handled within the generating case or here. Current default is to clear everything"
            n181 = call <vilib>:"Simple Error Handler.vi"("error in (no error)"=w74) -> ("error out"=w73:errorcluster)  [unwired: 4 in, 4 out]
            n182 = call <vilib>:"Clear Errors.vi"("error in (no error)"=w73) -> ("error out"=w72:errorcluster)  [unwired: 6 in]
          }
        }
      }
      n183 = Unregister For Events(event registration refnum=w57, error in=w56) -> (error out=w53:errorcluster)
      n184 = call <vilib>:"Simple Error Handler.vi"("error in (no error)"=w53) -> ()  [unwired: 4 in, 5 out]
    }
    frame Error {
    }
  }
